vi "GetPanelUI.vi"(8 "error in (no error)":errorcluster, 11 "object in":refnum<class "Template_CFG.lvclass">) -> (0 "error out":errorcluster, 2 "VI Refnum":refnum<vi>, 3 "object out":refnum<class "Template_CFG.lvclass">)   [LabVIEW 2021, in "Template-Channels.lvlib" / "Template_CFG.lvclass"]
uses:
  Template_CFG.lvclass
  Template_CFG.lvclass/Template_CFG.ctl
  TemplatePanel.vi
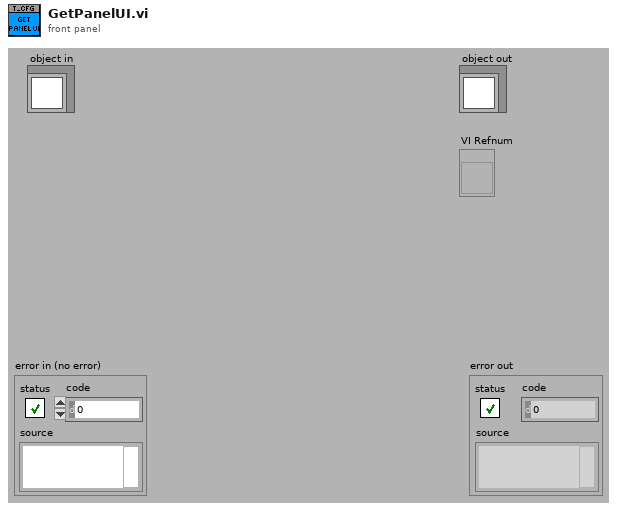
[diagram p1: front panel]
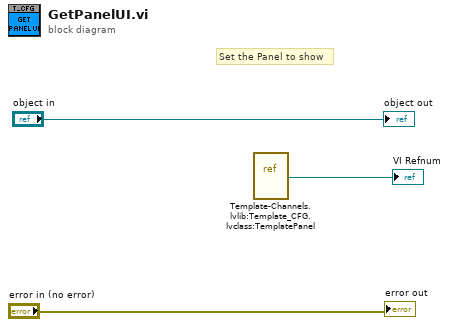
[diagram p0: block diagram]
diagram:
  # "Set the Panel to show"
  n1 = vi-ref "Template-Channels.lvlib:Template_CFG.lvclass:TemplatePanel.vi"() -> (→"VI Refnum":refnum<vi>)
  "error out" <- "error in (no error)"
  "object out" <- "object in"
